vi "modify channel test.vi"() -> (0 "no err":errorcluster, 3 "mod success":bool)   [LabVIEW 2014, in "Scan Engine tests.lvlib"]
uses:
  Scan Engine tests.lvlib
  <vilib>/NI/Tag Bus Module Framework/channel/TBM channel.lvclass/TBM channel.ctl
  <vilib>/NI/Tag Bus Module Framework/channel/channel classification.ctl
  <vilib>/NI/Tag Bus/tag/tag descriptor.lvclass/tag descriptor.ctl
  <vilib>/NI/Tag Bus Module Framework/channel/Read channel classification.vi
  <vilib>/NI/Tag Bus Module Framework/channel/Write channel classification.vi
  configuration/Scan Engine configuration.lvclass
  <vilib>/NI/Tag Bus Module Framework/channel/TBM channel.lvclass
  <vilib>/NI/Tag Bus/tag/tag descriptor.lvclass
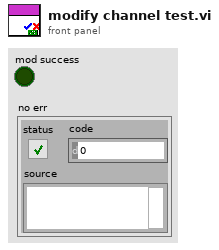
[diagram p1: front panel]
types:
  T1 = typedef "Scan Engine configuration.lvclass/Line.ctl" = cluster{"channel":refnum<class "TBM channel.lvclass">, "Tag":string}
  T2 = typedef "TBM channel.lvclass/channel classification.ctl" = enum16{"input data", "output data", "processing parameter", "processing result"}
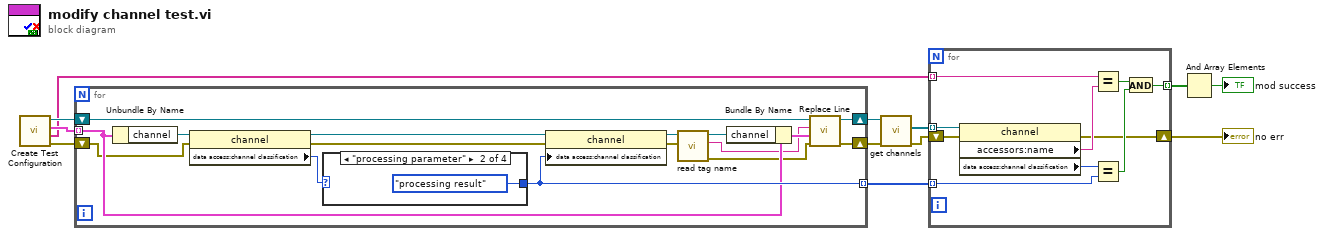
[diagram p0: block diagram]
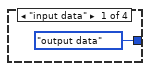
[diagram p2: hidden frame]
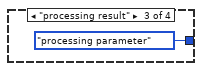
[diagram p3: hidden frame]
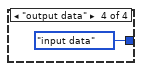
[diagram p4: hidden frame]
diagram:
  n1 = call "Create Test Configuration.vi"() -> ("error out"=w4:errorcluster, "Names"=w3:string[], "Line Array"=w5:T1[], "module"=w6:refnum<class "Scan Engine configuration.lvclass">)  [unwired: 6 in, 2 out]
  n2 = for {
    shift-right: [w21] -> w11
    shift-left: w6 -> [w20]
    shift-right: [w22] -> w2
    shift-left: w4 -> [w12]
    tunnel: w5 -> [w19] mode=indexing
    tunnel: [w24] -> w7 mode=indexing
    n3 = Unbundle By Name(w19) -> ("channel"=w23:refnum<class "TBM channel.lvclass">)
    n4 = property class="channel"(reference=w23, error in=w12) -> (reference out=w26:refnum<class "TBM channel.lvclass">, error out=w27:errorcluster, "data access:channel classification"=w25:T2)
    n5 = case shown="\"processing parameter\"" w25 {
      tunnel: [channel_classification."output data" ("channel classification") channel_classification."processing result" ("channel classification") channel_classification."processing parameter" ("channel classification") channel_classification."input data" ("channel classification")] -> w24
      frame "input data" {
      }
      frame "processing parameter" {
      }
      frame "processing result" {
      }
      frame "output data" {
      }
    }
    n6 = property class="channel"(reference=w26, error in=w27, "data access:channel classification"=w24) -> (reference out=w17:refnum<class "TBM channel.lvclass">, error out=w15:errorcluster)
    n7 = call <vilib>:"read tag name.vi"("error in"=w15, "system tag in"=w17) -> ("error out"=w14:errorcluster, "name"=w13:string, "system tag out"=w16:refnum<class "TBM channel.lvclass">)  [unwired: 7 in]
    n8 = Bundle By Name(cluster=w19, "channel"=w16) -> (w18:T1)
    n9 = call "Replace Line.vi"("error in"=w14, "New Line"=w18, "Line Name"=w13, "Scan Engine configuration in"=w20) -> ("error out"=w22:errorcluster, "Scan Engine configuration out"=w21:refnum<class "Scan Engine configuration.lvclass">)  [unwired: 5 in, 1 out]
  }
  n10 = call-dynamic "get channels.vi"("Scan Engine configuration in"=w11) -> ("channels"=w10:refnum<class "TBM channel.lvclass">[])  [unwired: 9 in, 1 out]
  n11 = for {
    tunnel: w10 -> [w40] mode=indexing
    tunnel: [w39] -> w9 mode=indexing
    tunnel: w7 -> [w38] mode=indexing
    tunnel: w3 -> [w35] mode=indexing
    shift-right: [w32] -> w1
    shift-left: w2 -> [w33]
    n12 = property class="channel"(reference=w40, error in=w33) -> (error out=w32:errorcluster, "accessors:name"=w36:string, "data access:channel classification"=w37:T2)  [unwired: 1 out]
    n13 = Equal?(x=w35, y=w36) -> (x = y?=w34:bool)
    n14 = Equal?(x=w37, y=w38) -> (x = y?=w41:bool)
    n15 = And(x=w34, y=w41) -> (x .and. y?=w39:bool)
  }
  "no err" <- w1
  n16 = And Array Elements(Boolean array=w9) -> (logical AND=→"mod success":bool)
